vi "Add Modifier to File Name.vi"(8 "error in (no error)":errorcluster, 9 "file name modifier":string, 10 "base path":path) -> (0 "error out":errorcluster, 2 "appended path":path)   [LabVIEW 2021, in "Logging.lvlib"]
doc: "Take 'base path' and append 'file name modifier' to the name part of the path, keeping the same exension. Returned in 'appended path'."
uses:
  Logging.lvlib
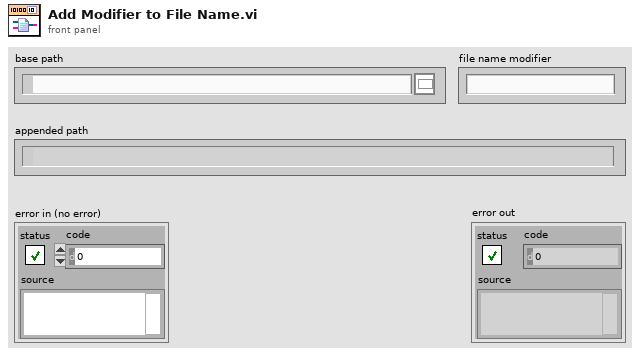
[diagram p1: front panel]
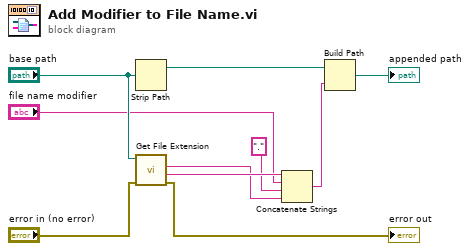
[diagram p0: block diagram]
diagram:
  n1 = Strip Path(path="base path") -> (stripped path=w7:path)  [unwired: 1 out]
  n2 = call <vilib>:"Get File Extension.vi"("error in (no error)"="error in (no error)", "file"="base path") -> ("error out"=→"error out":errorcluster, "filename without extension"=w8:string, "lowercase file extension"=w6:string)  [unwired: 5 in, 2 out]
  n3 = Concatenate Strings(w8, "file name modifier", "." ("string"), w6) -> (w9:string)
  n4 = Build Path(base path=w7, name or relative path=w9) -> (appended path=→"appended path":path)
